vi "update ring.vi"(7 "Interpret as Unicode (T)":bool, 8 "error in (no error)":errorcluster, 9 "Ring Texts":string[](array[string]), 11 "Ring Control Ref":refnum<vi>) -> (0 "error out":errorcluster, 3 "Ring Control Ref":refnum<vi>)   [LabVIEW 2019, in "Language Selection.lvlib"]
doc: "Uses \"Ring Texts\" to translate items of a Text ring control.\n- - -\nCopyright (c) 2026, Merecs Engineering GmbH"
uses:
  Language Selection.lvlib
panel:
  # "Connector Pane"
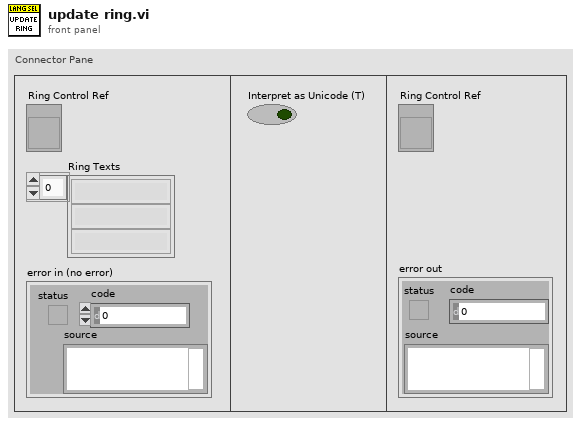
[diagram p1: front panel]
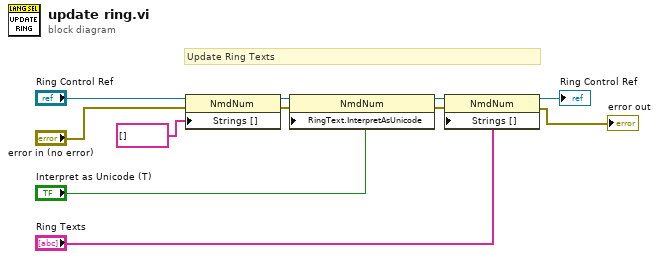
[diagram p0: block diagram]
diagram:
  # "Update Ring Texts"
  n1 = property class="NmdNum"(reference="Ring Control Ref", error in="error in (no error)", "Strings []"=string[] [] ("Strings [4]")) -> (reference out=w5:refnum<vi>, error out=w6:errorcluster)
  n2 = property class="NmdNum"(reference=w5, error in=w6, "RingText.InterpretAsUnicode"="Interpret as Unicode (T)") -> (reference out=w9:refnum<vi>, error out=w8:errorcluster)
  n3 = property class="NmdNum"(reference=w9, error in=w8, "Strings []"="Ring Texts") -> (reference out=→"Ring Control Ref":refnum<vi>, error out=→"error out":errorcluster)
